vi "Watchdog Configure.vi"(4 "error in (no error)":errorcluster, 5 "expiration actions":T1={"reset system"=FALSE, "restart LabVIEW Runtime"=FALSE, "occurrence"=FALSE, "trigger protocol"=enum."active high", "trigger line"=enum."none", "disable watchdog on VI exit"=TRUE}, 6 "timeout (1 sec)":dbl=1.0 format="%^.2e") -> (0 "error out":errorcluster, 1 "occurrence":refnum<k4>, 2 "timeout value returned (sec)":dbl format="%^.2e", 3 "watchdogID":u64=1 format="%.0x")   [LabVIEW 2025]
doc: "<p>Configures a new <a href=\"nihelplauncher://docs/csh?context=lvrt_lvrtconcepts_rt_watchdog\">watchdog object</a> with a <strong>timeout</strong> and <strong>expiration actions</strong>.</p>"
uses:
  Watchdog attribute enum.ctl
  Watchdog expiration actions.ctl
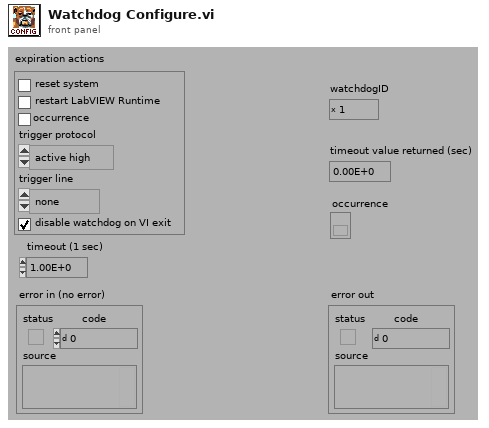
[diagram p1: front panel]
types:
  T1 = typedef "Watchdog expiration actions.ctl" = cluster{"reset system":bool, "restart LabVIEW Runtime":bool, "occurrence":bool, "trigger protocol":enum16{"active high", "active low", "open collector"}, "trigger line":enum16{"none", "line 0", "line 1", "line 2", "line 3", "line 4", "line 5", "line 6", "line 7", "SMB line 0"}, "disable watchdog on VI exit":bool}
  T2 = typedef "Watchdog attribute enum.ctl" = enum16{"current count", "hardware expire", "hardware ID", "hardware lock", "initial count", "instance", "resolution", "time step", "whack input source", "total timeout"}
  T3 = enum16{"none", "line 0", "line 1", "line 2", "line 3", "line 4", "line 5", "line 6", "line 7", "SMB line 0"}
  T4 = enum16{"active high", "active low", "open collector"}
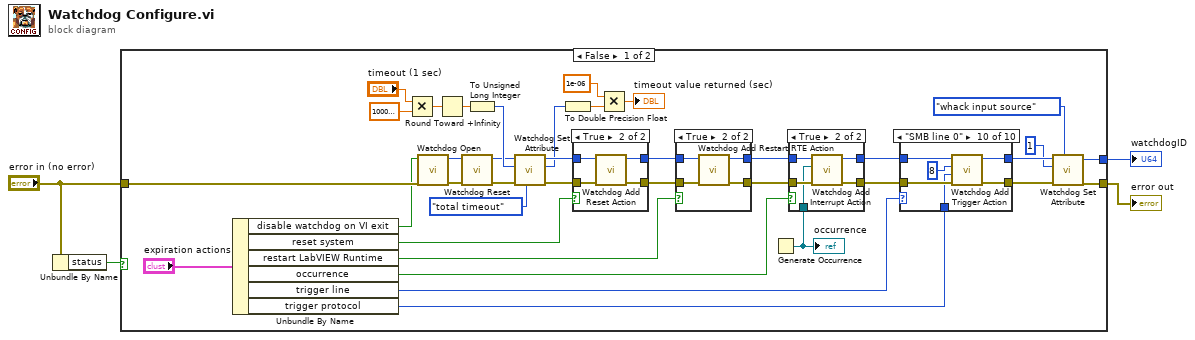
[diagram p0: block diagram]
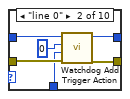
[diagram p6: hidden frame]
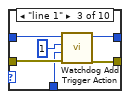
[diagram p7: hidden frame]
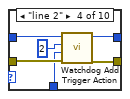
[diagram p8: hidden frame]
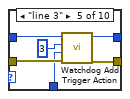
[diagram p9: hidden frame]
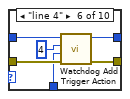
[diagram p10: hidden frame]
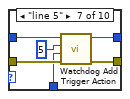
[diagram p11: hidden frame]
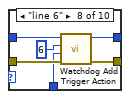
[diagram p12: hidden frame]
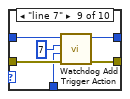
[diagram p13: hidden frame]
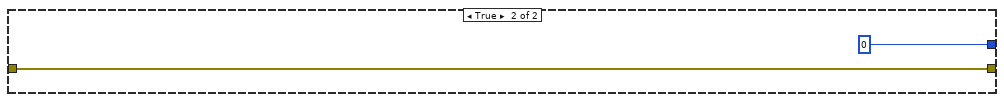
[diagram p14: hidden frame]
diagram:
  n1 = Unbundle By Name("error in (no error)") -> ("status"=w1:bool)
  n2 = case shown="False" w1 {
    tunnel: "error in (no error)" -> [w13 w118]
    tunnel: [w12 w118] -> w4
    tunnel: [w11 u32 0 ("watchdogID out")] -> w3
    frame False {
      n3 = Unbundle By Name("expiration actions") -> ("disable watchdog on VI exit"=w10:bool, "reset system"=w31:bool, "restart LabVIEW Runtime"=w8:bool, "occurrence"=w32:bool, "trigger line"=w41:T3, "trigger protocol"=w40:T4)
      n4 = Multiply(x="timeout (1 sec)", y=1000000.0) -> (x*y=w21:dbl)
      n5 = call "Watchdog Open.vi"("error in (no error)"=w13, "disable watchdog on VI exit (T)"=w10) -> ("error out"=w18:errorcluster, "watchdogID"=w15:u64)  [unwired: 4 in]
      n6 = Round Toward +Infinity(x=w21) -> (ceil(x): smallest int >= x=w22:dbl)
      n7 = call "Watchdog Reset.vi"("error in (no error)"=w18, "watchdogID in"=w15) -> ("error out"=w14:errorcluster, "watchdogID out"=w16:u64)  [unwired: 4 in]
      n8 = To Unsigned Long Integer(number=w22) -> (unsigned 32bit integer=w23:u32)
      n9 = call "Watchdog Set Attribute.vi"("attribute"=Watchdog_attribute_enum."total timeout", "error in (no error)"=w14, "attribute value"=w23, "watchdogID in"=w16) -> ("error out"=w30:errorcluster, "attribute value returned"=w25:u32, "watchdogID out"=w29:u64)  [unwired: 2 in]
      n10 = To Double Precision Float(number=w25) -> (double precision float=w26:dbl)
      n11 = case shown="True" w31 {
        tunnel: w29 -> [w49 w53]
        tunnel: [w49 w52] -> w9
        tunnel: [w48 w51] -> w5
        tunnel: w30 -> [w48 w50]
        frame False {
        }
        frame True {
          n12 = call "Watchdog Add Reset Action.vi"("error in (no error)"=w50, "watchdogID in"=w53) -> ("error out"=w51:errorcluster, "watchdogID out"=w52:u64)  [unwired: 4 in]
        }
      }
      n13 = Multiply(x=1e-06 ("y"), y=w26) -> (x*y=→"timeout value returned (sec)":dbl)
      n14 = case shown="True" w8 {
        tunnel: w9 -> [w43 w47]
        tunnel: [w43 w46] -> w7
        tunnel: [w42 w45] -> w6
        tunnel: w5 -> [w42 w44]
        frame False {
        }
        frame True {
          n15 = call "Watchdog Add Restart RTE Action.vi"("error in (no error)"=w44, "watchdogID in"=w47) -> ("error out"=w45:errorcluster, "watchdogID out"=w46:u64)  [unwired: 4 in]
        }
      }
      n16 = Generate Occurrence() -> (w33:refnum<k4>)
      "occurrence" <- w33
      n17 = case shown="True" w32 {
        tunnel: [w54 w58] -> w35
        tunnel: [w55 w57] -> w34
        tunnel: w6 -> [w55 w60]
        tunnel: w7 -> [w54 w59]
        tunnel: w33 -> [_ w56]
        frame False {
        }
        frame True {
          n18 = call "Watchdog Add Interrupt Action.vi"("error in (no error)"=w60, "Occurrence RefNum"=w56, "watchdogID in"=w59) -> ("error out"=w57:errorcluster, "watchdogID out"=w58:u64)  [unwired: 3 in]
        }
      }
      n19 = case shown="\"SMB line 0\"" w41 {
        tunnel: w35 -> [w62 w64 w70 w76 w82 w92 w98 w104 w110 w116]
        tunnel: [w62 w67 w73 w79 w85 w89 w95 w101 w107 w113] -> w39
        tunnel: [w61 w66 w72 w78 w84 w88 w94 w100 w106 w112] -> w38
        tunnel: w34 -> [w61 w65 w71 w77 w83 w91 w97 w103 w109 w115]
        tunnel: w40 -> [_ w63 w69 w75 w81 w87 w93 w99 w105 w111]
        frame "none", Default {
        }
        frame "line 0" {
          n20 = call "Watchdog Add Trigger Action.vi"("error in (no error)"=w65, "trigger protocol"=w63, "trigger ID"=u32 0, "watchdogID in"=w64) -> ("error out"=w66:errorcluster, "watchdogID out"=w67:u64)  [unwired: 2 in]
        }
        frame "line 1" {
          n21 = call "Watchdog Add Trigger Action.vi"("error in (no error)"=w71, "trigger protocol"=w69, "trigger ID"=u32 1, "watchdogID in"=w70) -> ("error out"=w72:errorcluster, "watchdogID out"=w73:u64)  [unwired: 2 in]
        }
        frame "line 2" {
          n22 = call "Watchdog Add Trigger Action.vi"("error in (no error)"=w77, "trigger protocol"=w75, "trigger ID"=u32 2, "watchdogID in"=w76) -> ("error out"=w78:errorcluster, "watchdogID out"=w79:u64)  [unwired: 2 in]
        }
        frame "line 3" {
          n23 = call "Watchdog Add Trigger Action.vi"("error in (no error)"=w83, "trigger protocol"=w81, "trigger ID"=u32 3, "watchdogID in"=w82) -> ("error out"=w84:errorcluster, "watchdogID out"=w85:u64)  [unwired: 2 in]
        }
        frame "line 4" {
          n24 = call "Watchdog Add Trigger Action.vi"("error in (no error)"=w91, "trigger protocol"=w87, "trigger ID"=u32 4, "watchdogID in"=w92) -> ("error out"=w88:errorcluster, "watchdogID out"=w89:u64)  [unwired: 2 in]
        }
        frame "line 5" {
          n25 = call "Watchdog Add Trigger Action.vi"("error in (no error)"=w97, "trigger protocol"=w93, "trigger ID"=u32 5, "watchdogID in"=w98) -> ("error out"=w94:errorcluster, "watchdogID out"=w95:u64)  [unwired: 2 in]
        }
        frame "line 6" {
          n26 = call "Watchdog Add Trigger Action.vi"("error in (no error)"=w103, "trigger protocol"=w99, "trigger ID"=u32 6, "watchdogID in"=w104) -> ("error out"=w100:errorcluster, "watchdogID out"=w101:u64)  [unwired: 2 in]
        }
        frame "line 7" {
          n27 = call "Watchdog Add Trigger Action.vi"("error in (no error)"=w109, "trigger protocol"=w105, "trigger ID"=u32 7, "watchdogID in"=w110) -> ("error out"=w106:errorcluster, "watchdogID out"=w107:u64)  [unwired: 2 in]
        }
        frame "SMB line 0" {
          n28 = call "Watchdog Add Trigger Action.vi"("error in (no error)"=w115, "trigger protocol"=w111, "trigger ID"=u32 8, "watchdogID in"=w116) -> ("error out"=w112:errorcluster, "watchdogID out"=w113:u64)  [unwired: 2 in]
        }
      }
      n29 = call "Watchdog Set Attribute.vi"("attribute"=Watchdog_attribute_enum."whack input source", "error in (no error)"=w38, "attribute value"=u32 1, "watchdogID in"=w39) -> ("error out"=w12:errorcluster, "watchdogID out"=w11:u64)  [unwired: 2 in, 1 out]
    }
    frame True {
    }
  }
  "error out" <- w4
  "watchdogID" <- w3
